vi "DriveMaxSpeed.vi"() -> (0 "Max Speed (m/sec)":dbl format="%#_13g", 3 "Max Speed (ft/sec)":dbl)   [LabVIEW 2023]
doc: "Constant variable for max speed of robot to use in calculations"
uses:
  <vilib>/Rock Robotics/WPI/ThirdParty/JAS_Junk/TrajLib/Trajectory_Library.lvlib
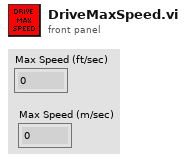
[diagram p1: front panel]
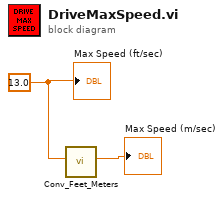
[diagram p0: block diagram]
diagram:
  w2 = 13.0
  n1 = call <vilib>:"Conv_Feet_Meters.vi"("Feet"=w2) -> ("Meters"=→"Max Speed (m/sec)":dbl)  [unwired: 10 in]
  "Max Speed (ft/sec)" <- w2
